vi "Make_RDDF(UTM).vi"() -> ()   [LabVIEW 2024]
uses:
  <vilib>/Utility/file.llb/Read Delimited Spreadsheet (DBL).vi
  <vilib>/Utility/file.llb/Write Delimited Spreadsheet (DBL).vi
panel:
  out "NMEA_Raw_Data":string
  out "Display_Long":dbl
  out "Display_Lat":dbl
  out "SOG(kph)":dbl format="%#_12g"
  in  "입력속도":dbl=5.0 format="%#_13g"
  out "UTM X(N) INS":dbl format="%#_13g"
  out "UTM Y(E) INS":dbl format="%#_13g"
  out "True_Heading":dbl format="%#_15g"
  in  "Stop":bool
  in  "file path (dialog if empty)":path caption="파일 경로(비었을 경우 대화 상자 창)"
  in  "dist.":dbl=0.2
  in  "Evt":bool
  out "XY 그래프":cluster{dbl[], dbl[]}[](graph)
  in  "File_Name(User):":string
  out "File_Name(Save):":string
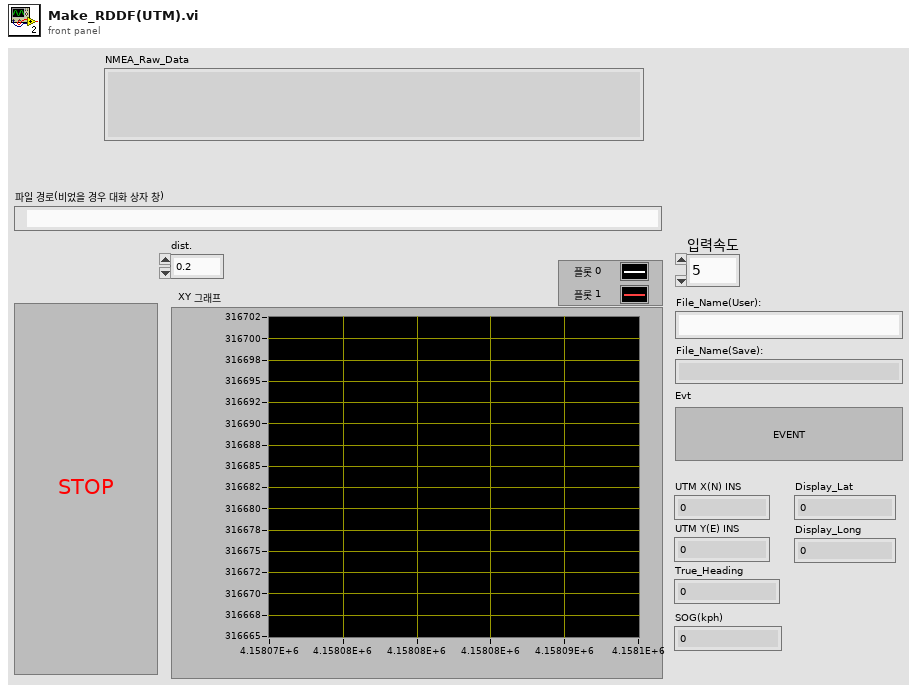
[diagram p1: front panel]
types:
  T1 = enum16{"Standard", "Buffered", "CRLF", "Immediate"}
  T2 = cluster{"oldest read timestamp":dbl, "latitude (deg)":dbl, "longitude (deg)":dbl, "ground speed (kph)":dbl, "true track angle (deg)":dbl, "altitude above mean sea level (m)":dbl}
  T3 = enum16{"open", "replace", "create", "open or create", "replace or create", "replace or create with confirmation"}
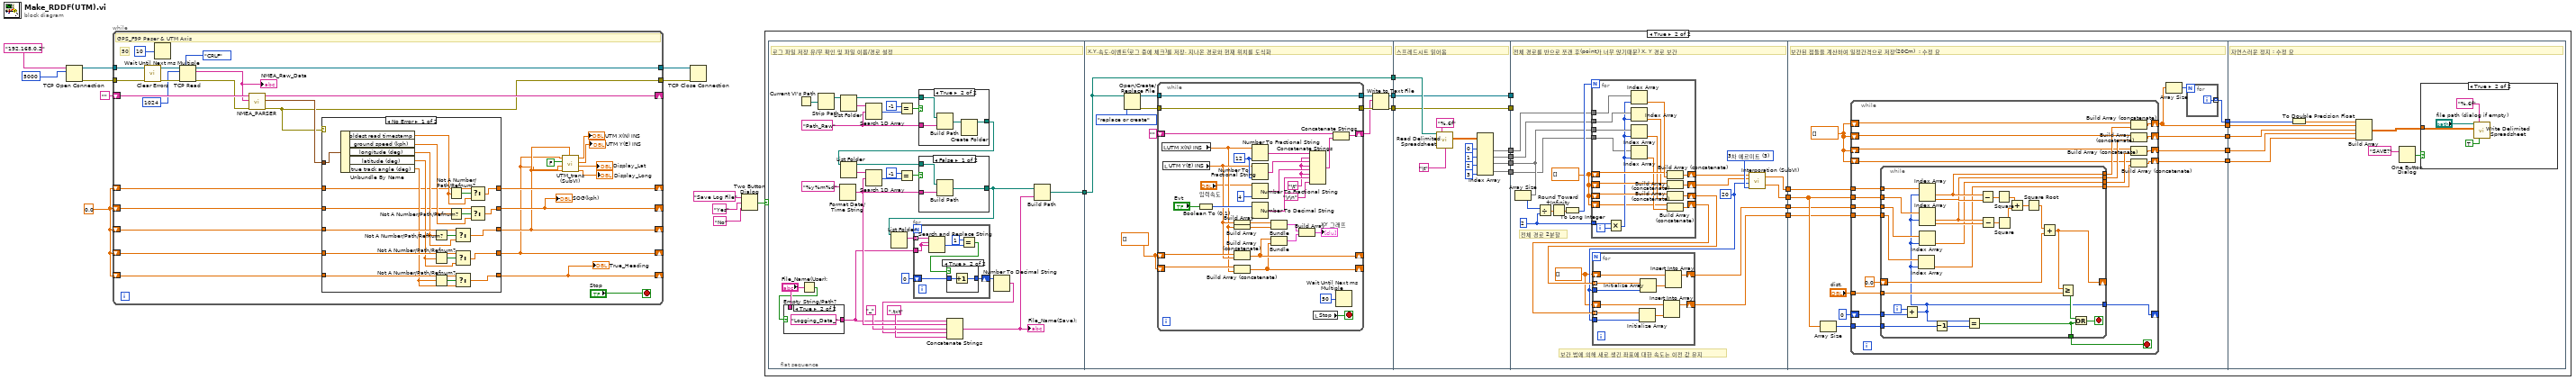
[diagram p0: block diagram]
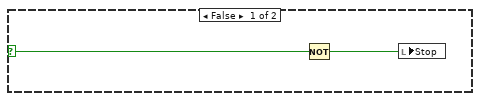
[diagram p3: hidden frame]
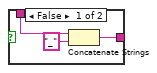
[diagram p4: hidden frame]
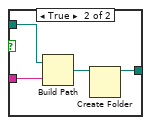
[diagram p6: hidden frame]
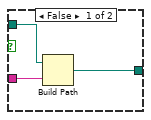
[diagram p7: hidden frame]
diagram:
  w7 = 0.0 ("x")
  n1 = TCP Open Connection(address="192.168.0.2", remote port or service name=u16 5000) -> (connection ID=w4:refnum<k5>, error out=w3:errorcluster)  [unwired: 3 in]
  n2 = while {
    tunnel: [w37] -> w6
    shift-right: [w38] -> _
    shift-left: "" -> [w40]
    shift-right: [w29] -> _
    shift-left: w7 -> [w36]
    shift-right: [w22] -> _
    shift-left: w7 -> [w35]
    shift-right: [w21] -> _
    shift-left: w7 -> [w34]
    shift-right: [w26] -> _
    shift-left: w7 -> [w33]
    shift-right: [w30] -> _
    shift-left: w7 -> [w32]
    tunnel: [w18] -> w5
    tunnel: w4 -> [w17]
    tunnel: w3 -> [w16]
    stop <- "Stop" stop-if-true
    # "50"
    # "GPS_F9P Paser & UTM Axis"
    n3 = call <vilib>:"Clear Errors.vi"("error in (no error)"=w16) -> ("error out"=w15:errorcluster)  [unwired: 5 in, 1 out]
    n4 = Wait Until Next ms Multiple(millisecond multiple=u32 10) -> ()  [unwired: 1 out]
    n5 = TCP Read(connection ID=w17, bytes to read=1024, error in (no error)=w15, 7:T1."CRLF" ("mode (standard)")) -> (connection ID out=w18:refnum<k5>, data out=w20:string, error out=w19:errorcluster)  [unwired: 1 in]
    "NMEA_Raw_Data" <- w20
    n6 = call "NMEA_PARSER.vi"("previous partial sentence"=w40, "sensor data"=w20, "error in (no error)"=w19) -> ("remaining partial sentence"=w38:string, "GPS data"=w39:T2, "error out"=w37:errorcluster)  [unwired: 5 in]
    n7 = case shown="No Error" w37 {
      tunnel: w39 -> [w62 _]
      tunnel: w35 -> [w58 w67]
      tunnel: w34 -> [w57 w66]
      tunnel: w33 -> [w56 w65]
      tunnel: [w52 w67] -> w22
      tunnel: [w51 w66] -> w21
      tunnel: [w50 w65] -> w26
      tunnel: w36 -> [w47 w64]
      tunnel: [w46 w64] -> w29
      tunnel: w32 -> [w43 w63]
      tunnel: [w42 w63] -> w30
      frame No Error {
        n8 = Unbundle By Name(w62) -> ("oldest read timestamp"=w44:dbl, "ground speed (kph)"=w48:dbl, "longitude (deg)"=w55:dbl, "latitude (deg)"=w54:dbl, "true track angle (deg)"=w53:dbl)
        n9 = Not A Number/Path/Refnum?(number/path/refnum=w55) -> (NaN/Path/Refnum?=w61:bool)
        n10 = Not A Number/Path/Refnum?(number/path/refnum=w54) -> (NaN/Path/Refnum?=w60:bool)
        n11 = Not A Number/Path/Refnum?(number/path/refnum=w53) -> (NaN/Path/Refnum?=w59:bool)
        n12 = Not A Number/Path/Refnum?(number/path/refnum=w44) -> (NaN/Path/Refnum?=w45:bool)
        n13 = Not A Number/Path/Refnum?(number/path/refnum=w48) -> (NaN/Path/Refnum?=w49:bool)
        n14 = Select(t=w58, s=w61, f=w55) -> (s? t:f=w52:dbl)
        n15 = Select(t=w57, s=w60, f=w54) -> (s? t:f=w51:dbl)
        n16 = Select(t=w56, s=w59, f=w53) -> (s? t:f=w50:dbl)
        n17 = Select(t=w43, s=w45, f=w44) -> (s? t:f=w42:dbl)
        n18 = Select(t=w47, s=w49, f=w48) -> (s? t:f=w46:dbl)
      }
      frame Error {
        # "Invalid data points."
      }
    }
    "SOG(kph)" <- w29
    "True_Heading" <- w26
    n19 = call "UTM_trans (SubVI).vi"("Long_Deg"=w22, "long"=w22, "lat"=w21, "East?West?"=FALSE, "Lat_Deg"=w21) -> ("Display_Long"=→"Display_Long":dbl, "Display_Lat"=→"Display_Lat":dbl, "UTM_Y(Northing)"=→"UTM Y(E) INS":dbl, "UTM_X(Easting)"=→"UTM X(N) INS":dbl)
  }
  n20 = TCP Close Connection(connection ID=w5, error in (no error)=w6) -> ()  [unwired: 1 in, 2 out]
  n21 = Two Button Dialog(message="Save Log File" ("메시지"), 1:"No" ("거짓 버튼 이름(\"취소\")"), 2:"Yes" ("참 버튼 이름(\"확인\")")) -> (T button?=w9:bool)
  n22 = case shown="True" w9 {
    selector: w9 -> [w69 _]
    frame False {
      n23 = Not(x=w69) -> (.not. x?=w68:bool)
      n24 = local write "Stop"(w68) -> ()
    }
    frame True {
      n25 = flat-sequence {
        tunnel: [w116] -> w88
        tunnel: w88 -> [w148]
        tunnel: [w148] -> w87
        tunnel: [w147] -> w86
        tunnel: [w146] -> w85
        tunnel: w87 -> [w198]
        tunnel: w86 -> [w194]
        tunnel: w85 -> [w195]
        tunnel: [w195] -> w83
        tunnel: [w194] -> w82
        tunnel: [w187] -> w81
        tunnel: [w188] -> w80
        tunnel: [w192] -> w79
        tunnel: [w185] -> w72
        tunnel: [w210] -> w84
        tunnel: w83 -> [_]
        tunnel: w82 -> [_]
        tunnel: w81 -> [w212]
        tunnel: w80 -> [w213]
        tunnel: w79 -> [w214]
        tunnel: [w206] -> w78
        tunnel: [w205] -> w77
        tunnel: w72 -> [w204]
        tunnel: [w199] -> w71
        tunnel: w84 -> [w256]
        tunnel: w78 -> [w258]
        tunnel: w77 -> [w257]
        tunnel: [w255] -> w76
        tunnel: [w254] -> w75
        tunnel: [w253] -> w74
        tunnel: [w252] -> w73
        tunnel: w71 -> [w251]
        tunnel: [w249] -> w70
        tunnel: w76 -> [w320]
        tunnel: w75 -> [w315]
        tunnel: w74 -> [w316]
        tunnel: w73 -> [w317]
        tunnel: w70 -> [w314]
        frame #0 {
          w111 = "Path_Raw" ("원소")
          # "로그 파일 저장 유/무 확인 및 파일 이름/경로 설정"
          n26 = Current VI's Path() -> (path=w115:path)
          n27 = Empty String/Path?(string/path="File_Name(User):") -> (empty?=w91:bool)
          n28 = case shown="True" w91 {
            tunnel: [w118 "Logging_Data_"] -> w95
            tunnel: "File_Name(User):" -> [w117 _]
            frame False {
              n29 = Concatenate Strings(w117, "_" ("문자열")) -> (w118:string)
            }
            frame True {
            }
          }
          n30 = Strip Path(path=w115) -> (stripped path=w114:path)  [unwired: 1 out]
          n31 = Format Date/Time String(time format string (%c)="%y%m%d" ("시간 포맷 문자열 (%c)")) -> (date/time string=w98:string)  [unwired: 2 in]
          n32 = List Folder(path=w114) -> (path out=w113:path, folder names=w110:string[])  [unwired: 3 in, 2 out]
          n33 = Search 1D Array(1D array=w110, element=w111) -> (index of element=w109:i32)  [unwired: 1 in]
          n34 = Equal?(x=-1 ("y"), y=w109) -> (x = y?=w112:bool)
          n35 = case shown="True" w112 {
            tunnel: w113 -> [w138 w143]
            tunnel: w111 -> [w139 w142]
            tunnel: [w140 w141] -> w101
            frame False {
              n36 = Build Path(base path=w138, name or relative path=w139) -> (appended path=w140:path)
            }
            frame True {
              n37 = Build Path(base path=w143, name or relative path=w142) -> (appended path=w144:path)
              n38 = Create Folder(path (use dialog)=w144) -> (created path=w141:path)  [unwired: 2 in, 2 out]
            }
          }
          n39 = List Folder(path=w101) -> (path out=w102:path, folder names=w104:string[])  [unwired: 3 in, 2 out]
          n40 = Search 1D Array(1D array=w104, element=w98) -> (index of element=w105:i32)  [unwired: 1 in]
          n41 = Equal?(x=-1 ("y"), y=w105) -> (x = y?=w103:bool)
          n42 = case shown="False" w103 {
            tunnel: w102 -> [w131 w136]
            tunnel: w98 -> [w132 w135]
            tunnel: [w133 w134] -> w90
            frame False {
              n43 = Build Path(base path=w131, name or relative path=w132) -> (appended path=w133:path)
            }
            frame True {
              n44 = Build Path(base path=w136, name or relative path=w135) -> (appended path=w137:path)
              n45 = Create Folder(path (use dialog)=w137) -> (created path=w134:path)  [unwired: 2 in, 2 out]
            }
          }
          n46 = List Folder(path=w90) -> (filenames=w100:string[])  [unwired: 3 in, 3 out]
          n47 = for {
            tunnel: w100 -> [w127] mode=indexing
            shift-right: [w122] -> w94
            shift-left: 0 -> [w123]
            tunnel: w95 -> [w121]
            n48 = Search and Replace String(input string=w127, search string=w121, replace string=w121) -> (number of replacements=w125:i32)  [unwired: 5 in, 3 out]
            n49 = Equal?(x=1, y=w125) -> (x = y?=w124:bool)
            n50 = case shown="True" w124 {
              tunnel: w123 -> [w128 w130]
              tunnel: [w128 w129] -> w122
              frame False {
              }
              frame True {
                n51 = Increment(x=w130) -> (x+1=w129:i32)
              }
            }
          }
          n52 = Number To Decimal String(number=w94) -> (decimal integer string=w93:string)  [unwired: 1 in]
          n53 = Concatenate Strings(w95, w98, "_" ("문자열"), w93, ".txt" ("문자열")) -> (w89:string)
          "File_Name(Save):" <- w89
          n54 = Build Path(base path=w90, name or relative path=w89) -> (appended path=w116:path)
        }
        frame #1 {
          w145 = dbl[] []
          # "X,Y,속도,이벤트(로그 중에 체크)를 저장, 지나온 경로와 현재 위치를 도식화"
          n55 = Open/Create/Replace File(file path (use dialog)=w148, operation (0:open)=T3."replace or create" ("동작(0:open)")) -> (refnum out=w153:refnum<file>, error out=w154:errorcluster)  [unwired: 4 in, 1 out]
          n56 = while {
            tunnel: w154 -> [w179]
            tunnel: w153 -> [w180]
            tunnel: [w180] -> w151
            tunnel: [w179] -> w152
            shift-right: [w164] -> w150
            shift-left: "" -> [w166]
            shift-right: [w160] -> _
            shift-left: w145 -> [w171]
            shift-right: [w159] -> _
            shift-left: w145 -> [w170]
            stop <- w178 stop-if-true
            w173 = "\t"
            w184 = i16 12 ("정밀도(6)")
            n57 = local read "UTM X(N) INS"() -> (w157:dbl)
            n58 = local read "UTM Y(E) INS"() -> (w158:dbl)
            n59 = Boolean To (0,1)(Boolean="Evt") -> (0, 1=w181:i16)
            n60 = Build Array(w158) -> (w169:dbl[])
            n61 = Build Array(w157) -> (w168:dbl[])
            n62 = Build Array (concatenate)(w171, w158) -> (w160:dbl[])
            n63 = Build Array (concatenate)(w170, w157) -> (w159:dbl[])
            n64 = Number To Fractional String(number=w157, precision (6)=w184) -> (F-format string=w177:string)  [unwired: 2 in]
            n65 = Number To Fractional String(number=w158, precision (6)=w184) -> (F-format string=w176:string)  [unwired: 2 in]
            n66 = Number To Fractional String(number="입력속도", precision (6)=i16 4 ("정밀도(6)")) -> (F-format string=w175:string)  [unwired: 2 in]
            n67 = Number To Decimal String(number=w181) -> (decimal integer string=w174:string)  [unwired: 1 in]
            n68 = Bundle(w169, w168) -> (w161:cluster{dbl[], dbl[]})  [unwired: 1 in]
            n69 = Bundle(w160, w159) -> (w162:cluster{dbl[], dbl[]})  [unwired: 1 in]
            n70 = Build Array(w161, w162) -> (→"XY 그래프":cluster{dbl[], dbl[]}[])
            n71 = Concatenate Strings(w177, w173, w176, w173, w175, w173, w174, "\r\n") -> (w165:string)
            n72 = local read "Stop"() -> (w178:bool)
            n73 = Concatenate Strings(w166, w165) -> (w164:string)
            n74 = Wait Until Next ms Multiple(millisecond multiple=u32 50 ("ms 배수")) -> ()  [unwired: 1 out]
          }
          n75 = Write to Text File(file (use dialog)=w151, text=w150, error in=w152) -> (refnum out=w146:refnum<file>, error out=w147:errorcluster)  [unwired: 1 in, 1 out]
        }
        frame #2 {
          # "스프레드시트 읽어옴"
          n76 = call-poly <vilib>:"Read Delimited Spreadsheet.vi"("file path (dialog if empty)"=w198, "format (%.3f)"="%.6f", "delimiter (\\t)"="\t") -> ("all rows"=w193:dbl[][])  [unwired: 7 in, 5 out]
          n77 = Index Array(array=w193, index (col) #1=0 ("비활성화된 인덱스 (열)"), index (col) #2=1 ("인덱스 (열)"), index (col) #3=2 ("인덱스 (열)"), index (col) #4=3 ("인덱스 (열)")) -> (element #1=w192:dbl[], element #2=w188:dbl[], element #3=w187:dbl[], element #4=w185:dbl[])  [unwired: 4 in]
        }
        frame #3 {
          w209 = 3 items=["최근접", "선형", "스플라인", "3차 에르미트", "라그랑지"] ("method")
          w200 = dbl[] []
          w201 = 20 ("Interpolation factor (n)")
          w203 = dbl[] []
          w215 = 2
          # "보간 법에 의해 새로 생긴 좌표에 대한 속도는 이전 값 유지"
          # "전체 경로 2분할"
          # "전체 경로를 반으로 쪼갠 후(point가 너무 많기때문) X, Y 경로 보간"
          n78 = Array Size(array=w212) -> (size(s)=w219:i32)
          n79 = Divide(x=w219, y=w215) -> (x/y=w218:dbl)
          n80 = Round Toward +Infinity(x=w218) -> (ceil(x): smallest int >= x=w217:dbl)
          n81 = To Long Integer(number=w217) -> (32bit integer=w216:i32)
          n82 = for {
            N: w216 -> [_]
            tunnel: w215 -> [w247]
            tunnel: w214 -> [w246]
            tunnel: w213 -> [w245]
            tunnel: w212 -> [w244]
            shift-right: [w241] -> w208
            shift-left: w203 -> [w242]
            shift-right: [w240] -> w207
            shift-left: w203 -> [w239]
            shift-right: [w233] -> w211
            shift-left: w203 -> [w238]
            tunnel: w204 -> [w234]
            shift-right: [w230] -> w202
            shift-left: w203 -> [w231]
            i -> [w248]
            n83 = Multiply(x=w247, y=w248) -> (x*y=w235:i32)
            n84 = Index Array(array=w246, index=w235) -> (element=w243:dbl)
            n85 = Index Array(array=w245, index=w235) -> (element=w237:dbl)
            n86 = Index Array(array=w244, index=w235) -> (element=w236:dbl)
            n87 = Index Array(array=w234, index=w235) -> (element=w232:dbl)
            n88 = Build Array (concatenate)(w242, w243) -> (w241:dbl[])
            n89 = Build Array (concatenate)(w239, w237) -> (w240:dbl[])
            n90 = Build Array (concatenate)(w238, w236) -> (w233:dbl[])
            n91 = Build Array (concatenate)(w231, w232) -> (w230:dbl[])
          }
          n92 = for {
            tunnel: w211 -> [w229] mode=indexing
            tunnel: w201 -> [w228]
            shift-right: [w227] -> w210
            shift-left: w200 -> [w226]
            tunnel: w202 -> [w223] mode=indexing
            tunnel: w201 -> [w222]
            shift-right: [w220] -> w199
            shift-left: w200 -> [w221]
            n93 = Initialize Array(w223, w222) -> (w225:dbl[])
            n94 = Initialize Array(w229, w228) -> (w224:dbl[])
            n95 = Insert Into Array(array=w221, new element=w225) -> (w220:dbl[])  [unwired: 1 in]
            n96 = Insert Into Array(array=w226, new element=w224) -> (w227:dbl[])  [unwired: 1 in]
          }
          n97 = call "Interporation (SubVI).vi"("method"=w209, "Sample"=w201, "Y_long"=w207, "X_lat"=w208) -> ("Y_long"=w205:dbl[], "X_lat"=w206:dbl[])
        }
        frame #4 {
          w250 = dbl[] []
          # "보간된 점들을 계산하여 일정간격으로 저장(20Cm)  : 수정 요"
          n98 = Array Size(array=w257) -> (size(s)=w260:i32)
          n99 = while {
            tunnel: "dist." -> [w282]
            tunnel: w258 -> [w285]
            tunnel: w257 -> [w284]
            tunnel: w256 -> [w276]
            shift-right: [w271] -> _
            shift-left: 0 -> [w281]
            shift-right: [w268] -> w252
            shift-left: w250 -> [w277]
            shift-right: [w270] -> w253
            shift-left: w250 -> [w278]
            shift-right: [w269] -> w254
            shift-left: w250 -> [w274]
            tunnel: w260 -> [w273]
            tunnel: w251 -> [w267]
            shift-right: [w265] -> w249
            shift-left: w250 -> [w264]
            stop <- w272 stop-if-true
            n100 = while {
              tunnel: w285 -> [w312]
              tunnel: w284 -> [w311]
              shift-right: [w301] -> _
              shift-left: 0.0 -> [w302]
              tunnel: w282 -> [w300]
              tunnel: [w286] -> w271
              tunnel: w281 -> [w298]
              tunnel: [w297] -> w280
              tunnel: [w296] -> w279
              tunnel: w276 -> [w295]
              tunnel: [w294] -> w275
              tunnel: w273 -> [w293]
              tunnel: [w290] -> w272
              tunnel: w267 -> [w287]
              tunnel: [w288] -> w266
              i -> [w299]
              stop <- w292 stop-if-true
              n101 = Add(x=w299, y=w298) -> (x+y=w286:i32)
              n102 = Index Array(array=w287, index=w286) -> (element=w288:dbl)
              n103 = Index Array(array=w312, index #1=w286) -> (element #1=w297:dbl, element #2=w310:dbl)  [unwired: 1 in]
              n104 = Index Array(array=w311, index #1=w286) -> (element #1=w296:dbl, element #2=w309:dbl)  [unwired: 1 in]
              n105 = Index Array(array=w295, index=w286) -> (element=w294:dbl)
              n106 = Decrement(x=w293) -> (x-1=w289:i32)
              n107 = Equal?(x=w286, y=w289) -> (x = y?=w290:bool)
              n108 = Subtract(x=w297, y=w310) -> (x-y=w308:dbl)
              n109 = Subtract(x=w296, y=w309) -> (x-y=w307:dbl)
              n110 = Square(x=w308) -> (x^2=w306:dbl)
              n111 = Square(x=w307) -> (x^2=w305:dbl)
              n112 = Add(x=w306, y=w305) -> (x+y=w304:dbl)
              n113 = Square Root(x=w304) -> (sqrt(x)=w303:dbl)
              n114 = Add(x=w303, y=w302) -> (x+y=w301:dbl)
              n115 = Greater Or Equal?(x=w301, y=w300) -> (x >= y?=w291:bool)
              n116 = Or(x=w291, y=w290) -> (x .or. y?=w292:bool)
            }
            n117 = Build Array (concatenate)(w277, w280) -> (w268:dbl[])
            n118 = Build Array (concatenate)(w278, w279) -> (w270:dbl[])
            n119 = Build Array (concatenate)(w274, w275) -> (w269:dbl[])
            n120 = Build Array (concatenate)(w264, w266) -> (w265:dbl[])
          }
          n121 = Array Size(array=w252) -> (size(s)=w259:i32)
          n122 = for {
            N: w259 -> [_]
            tunnel: [w263] -> w255 mode=indexing
            i -> [w263]
          }
        }
        frame #5 {
          # "자연스러운 정지 : 수정 요"
          n123 = To Double Precision Float(number=w320) -> (double precision float=w313:dbl[])
          n124 = Build Array(w313, w317, w316, w315, w314) -> (w321:dbl[][])
          n125 = One Button Dialog(message="SAVE?") -> (true=w319:bool)  [unwired: 1 in]
          n126 = case shown="True" w319 {
            tunnel: w321 -> [_ w325]
            frame False {
            }
            frame True {
              n127 = call-poly <vilib>:"Write Delimited Spreadsheet.vi"("file path (dialog if empty)"="file path (dialog if empty)", "format (%.3f)"="%.6f", "2D data"=w325, "transpose? (no:F)"=TRUE) -> ()  [unwired: 10 in, 2 out]
            }
          }
        }
      }
    }
  }
